vi "LinearSystem_CalculateX.vi"(8 "dT_Seconds":dbl, 9 "ClampedU":T1, 10 "X":T1, 11 "Linearsystem":T2) -> (0 "Error":bool, 3 "outX":T1)   [LabVIEW 2019, in "Trajectory_Library.lvlib"]
doc: "Computes the new x given the old x and the control input.\n \nThis is used by state observers directly to run updates based on state estimate.\n\nInputs:\n - LinearSystem -- system data cluster\n - x -- The current state.\n - clampedU -- The control input.\n - dtSeconds -- Timestep for model update.\n\nOutputs:\n - outX -- the updated x.\n - error -- If TRUE, an error occured"
uses:
  Trajectory_Library.lvlib
  <vilib>/Analysis/NI_AALBase.lvlib
  <vilib>/Analysis/baseanly.llb/Real A x B.vi
  <vilib>/Analysis/Matrix/NI_Matrix.lvlib
  <vilib>/Analysis/Matrix/Numeric/Add/Add - RM,RM.vi
  TypeDef/LINEAR_SYSTEM.ctl
  <vilib>/Analysis/Matrix/Datatypes/RealMatrix.ctl
panel:
  # "<States,States>"
  # "<States,Inputs>"
  # "<Outputs,States>"
  # "<Outputs,Inputs>"
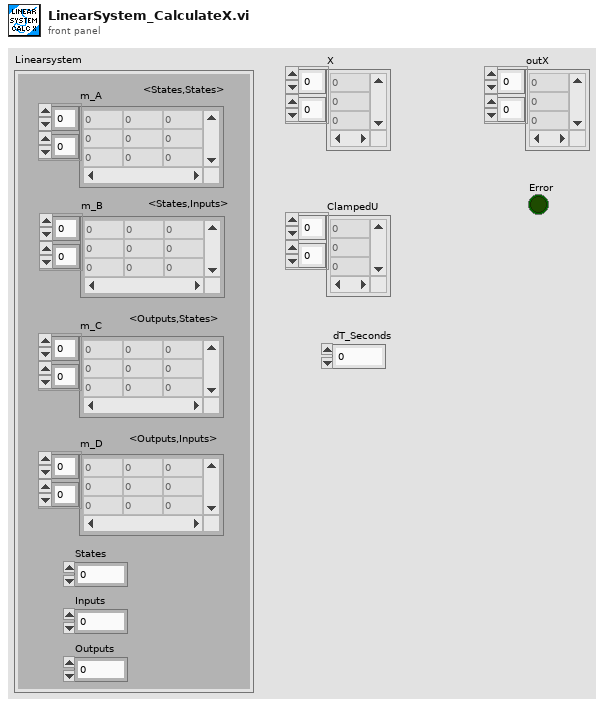
[diagram p1: front panel]
types:
  T1 = typedef "NI_Matrix.lvlib/RealMatrix.ctl" = dbl[][]
  T2 = typedef "Trajectory_Library.lvlib/LINEAR_SYSTEM.ctl" = cluster{"m_A":T1, "m_B":T1, "m_C":T1, "m_D":T1, "States":i32, "Inputs":i32, "Outputs":i32}
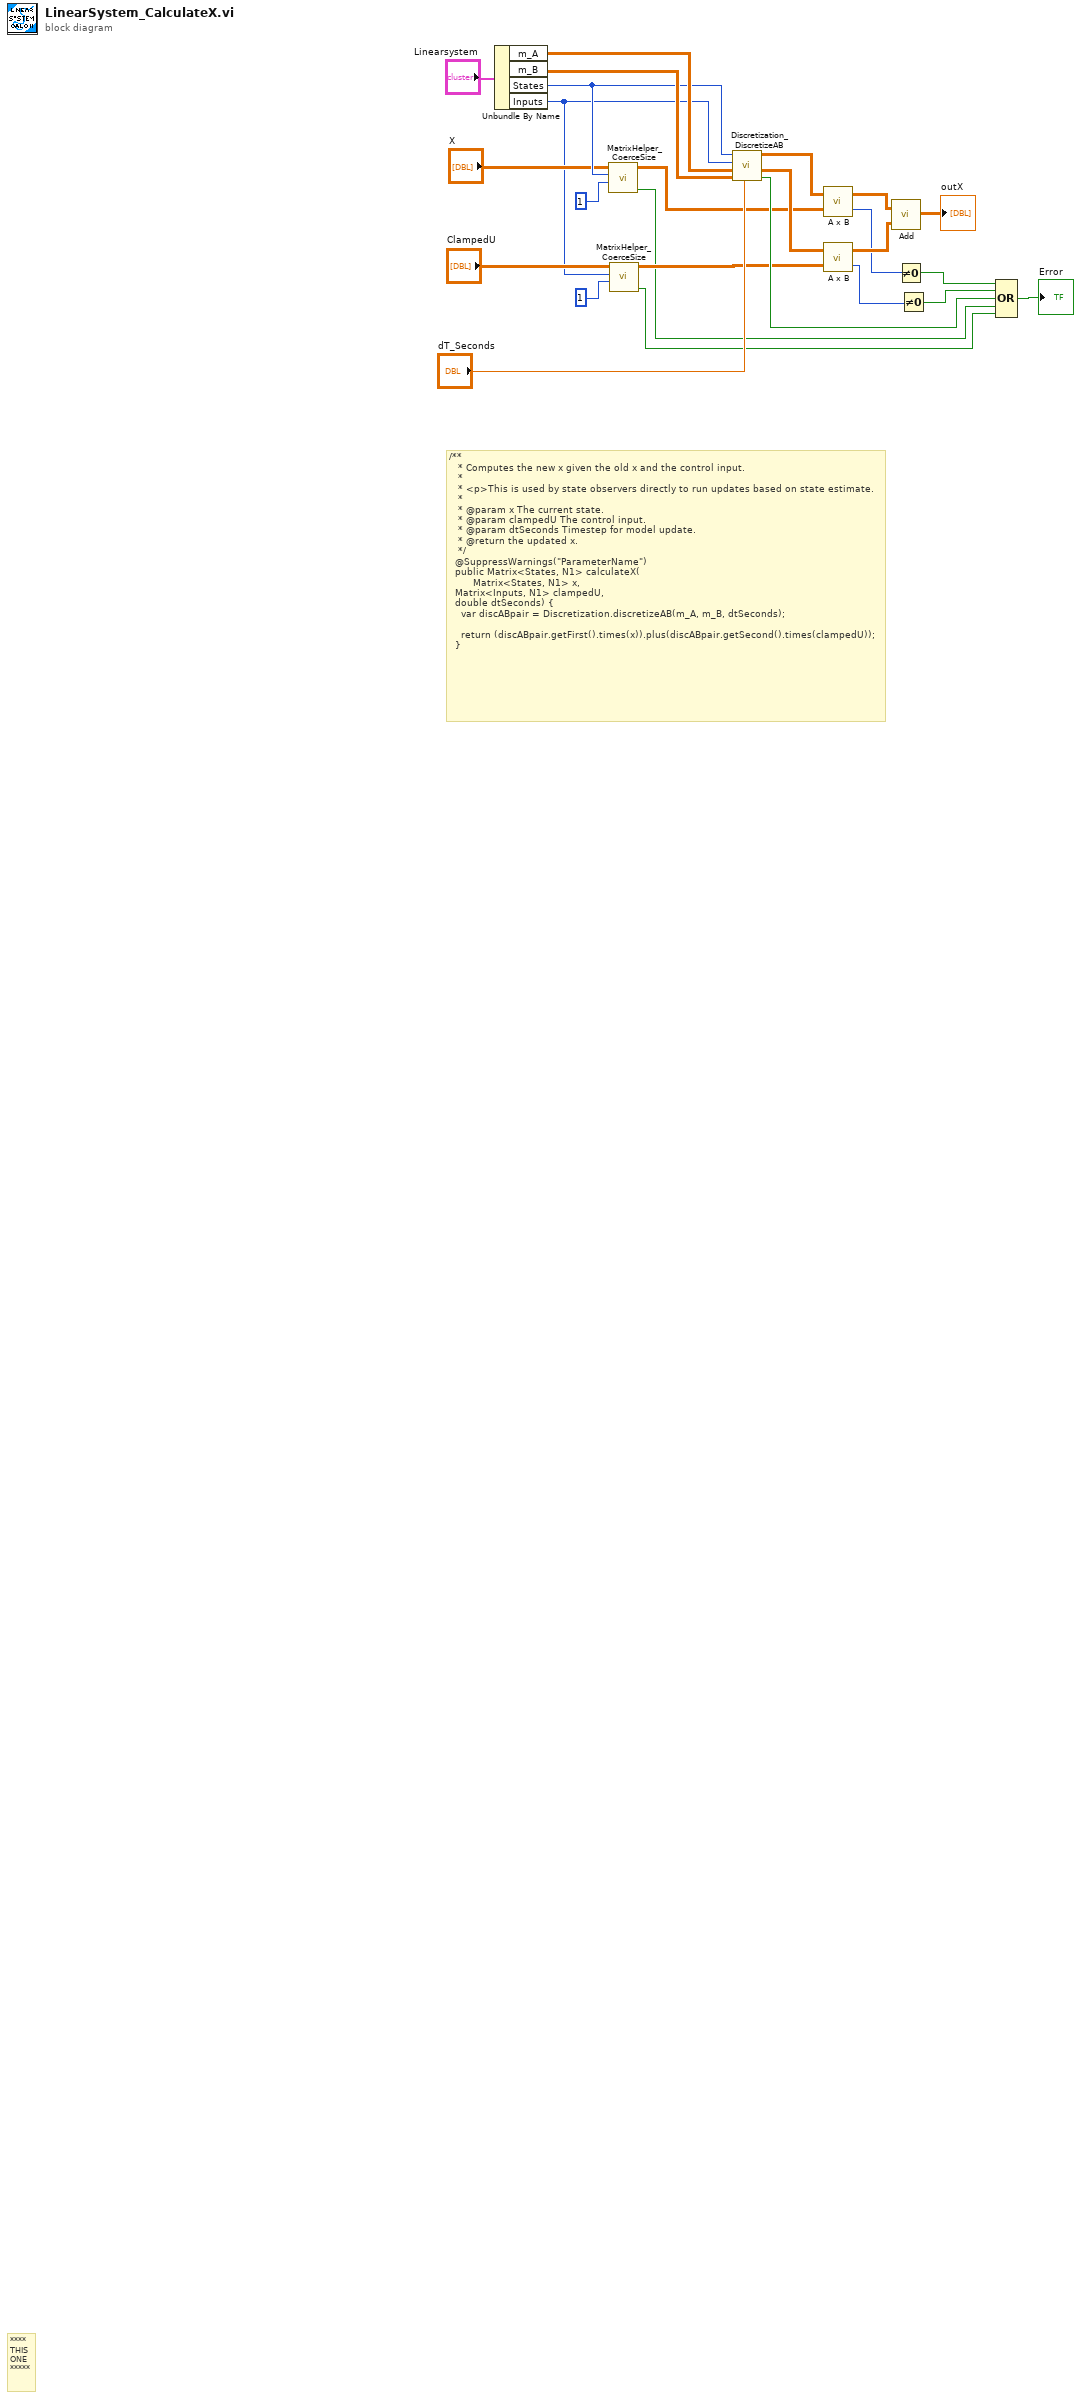
[diagram p0: block diagram]
diagram:
  # "/**\n   * Computes the new x given the old x and the control input.\n   *\n   * <p>This is used by state observers directly to run updates based on state estimate.\n   *\n   * @param x The current state.\n   * @param clampedU The control input.\n   * @param dtSeconds Timestep for model update.\n   * @return the updated x.\n   */\n  @SuppressWarnings(\"ParameterName\")\n  public Matrix<States, N1> calculateX(\n      \t\tMatrix<States, N1> x, \n\t\tMatrix<Inputs, N1> clampedU, \n\t\tdouble dtSeconds) {\n    var discABpair = Discretization.discretizeAB(m_A, m_B, dtSeconds);\n\n    return (discABpair.getFirst().times(x)).plus(discABpair.getSecond().times(clampedU));\n  }"
  # "****\nTHIS\nONE\n*****"
  n1 = Unbundle By Name("Linearsystem") -> ("m_A"=w24:T1, "m_B"=w23:T1, "States"=w10:i32, "Inputs"=w5:i32)
  n2 = call "MatrixHelper_CoerceSize.vi"("Columns"=1 ("number of columns"), "Rows"=w10, "input matrix"="X") -> ("Coerced"=w2:bool, "output matrix"=w7:T1)  [unwired: 7 in]
  n3 = call "MatrixHelper_CoerceSize.vi"("Columns"=1 ("number of columns"), "Rows"=w5, "input matrix"="ClampedU") -> ("Coerced"=w1:bool, "output matrix"=w3:T1)  [unwired: 7 in]
  n4 = call "Discretization_DiscretizeAB.vi"("dT_Seconds"="dT_Seconds", "ContB"=w23, "ContA"=w24, "Inputs"=w5, "States"=w10) -> ("Error"=w14:bool, "DiscB"=w20:T1, "DiscA"=w21:T1)  [unwired: 4 in]
  n5 = call-poly <vilib>:"A x B.vi"("B"=w7, "A"=w21) -> ("error"=w12:i32, "A x B"=w19:T1)
  n6 = call-poly <vilib>:"A x B.vi"("B"=w3, "A"=w20) -> ("error"=w13:i32, "A x B"=w18:T1)
  n7 = call-poly <vilib>:"Add.vi"("Real Matrix B"=w18, "Real Matrix A"=w19) -> ("A + B"=→"outX":T1)
  n8 = Not Equal To 0?(x=w12) -> (x != 0?=w16:bool)
  n9 = Not Equal To 0?(x=w13) -> (x != 0?=w15:bool)
  n10 = Compound Arithmetic op=OR(w16, w15, w14, w2, w1) -> (→"Error":bool)
